vi "Init Events.vi"(8 "error in (no error)":errorcluster, 11 "TSEngine in":refnum<class "Engine.lvclass">) -> (0 "error out":errorcluster, 3 "TSEngine out":refnum<class "Engine.lvclass">, 4 "Event Reg":refnum<event-registration>, 6 "Events":T1)   [LabVIEW 2020, in "TSS.lvlib" / "Engine.lvclass"]
uses:
  Engine.lvclass
  Events.ctl
  Create VC Event Data.ctl
  Variable Container Type.ctl
  VariableContainer/Typedefs/Session Handle.ctl
  VariableContainer/VariableContainer.lvclass
  Create Report Event Data.ctl
  Execution/Typedefs/Session Handle.ctl
  Execution/Execution.lvclass
  Report/Typedefs/Session Handle.ctl
  Report/Report.lvclass
  Open Sequence File Event Data.ctl
  Data Types/File Load Options.ctl
  SequenceFile/Typedefs/Session Handle.ctl
  SequenceFile/SequenceFile.lvclass
  Session Notification.ctl
  Prepare Execution Event Data.ctl
  Execution/Execution Options.ctl
  Engine.lvclass/Engine.ctl
  TSS.lvlib
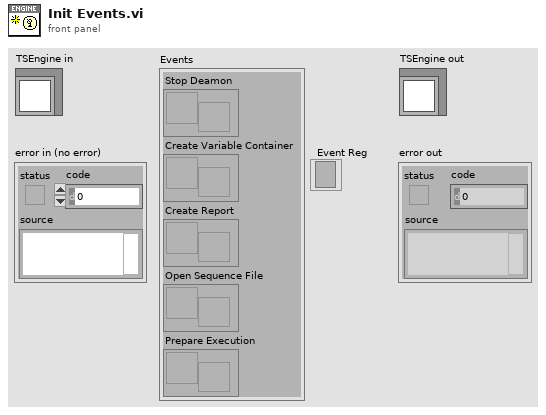
[diagram p1: front panel]
types:
  T1 = typedef "TSS.lvlib/Engine.lvclass/Events.ctl" = cluster{"Stop Deamon":refnum<user-event>, "Create Variable Container":refnum<user-event>, "Create Report":refnum<user-event>, "Open Sequence File":refnum<user-event>, "Prepare Execution":refnum<user-event>}
  T2 = typedef "TSS.lvlib/Engine.lvclass/Prepare Execution Event Data.ctl" = cluster{"Execution Options":T3, "Engine":refnum<data-value>, "Session Notifier":refnum<notifier>}
  T3 = typedef "TSS.lvlib/Execution.lvclass/Execution Options.ctl" = cluster{"Use Default Model":bool}
  T4 = typedef "TSS.lvlib/Engine.lvclass/Open Sequence File Event Data.ctl" = cluster{"File Path":path, "Load Options":T5, "Current Seq File (None)":T6, "Session Notifier":refnum<notifier>, "Engine":refnum<data-value>}
  T5 = typedef "TSS.lvlib/File Load Options.ctl" = cluster{"Use Search Dirs? (T)":bool, "Conflict as Error? (T)":bool, "Check Station Model? (F)":bool, "Preload Modules? (T)":bool, "Skip Load Callback? (F)":bool, "Reload if Loaded? (F)":bool}
  T6 = typedef "TSS.lvlib/SequenceFile.lvclass/Session Handle.ctl" = refnum<data-value>
  T7 = typedef "TSS.lvlib/Engine.lvclass/Create Report Event Data.ctl" = cluster{"Execution":T8, "Report Notifier":refnum<notifier>}
  T8 = typedef "TSS.lvlib/Execution.lvclass/Session Handle.ctl" = refnum<data-value>
  T9 = typedef "TSS.lvlib/Engine.lvclass/Create VC Event Data.ctl" = cluster{"Type":T10, "Notifier":refnum<notifier>}
  T10 = typedef "TSS.lvlib/Engine.lvclass/Variable Container Type.ctl" = enum16{"StationGlobals", "TemporaryGlobals", "NewPropertyObject"}
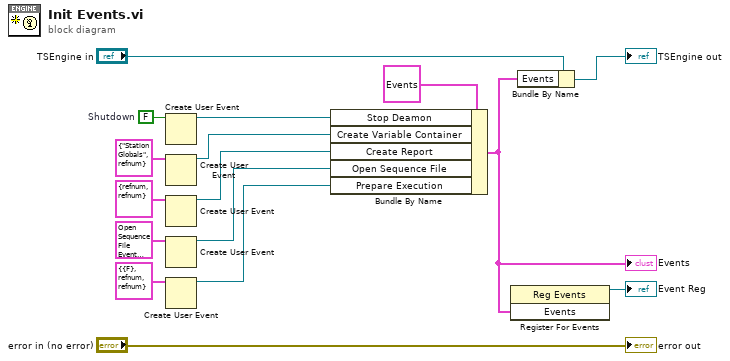
[diagram p0: block diagram]
diagram:
  w15 = FALSE  # Shutdown
  n1 = Create User Event(user event datatype=w15) -> (user event=w11:refnum<user-event>)  [unwired: 1 in, 1 out]
  n2 = Create User Event(user event datatype=T9 {"Type"=enum."StationGlobals", "Notifier"=refnum} ("Create VariableContainer Session")) -> (user event=w10:refnum<user-event>)  [unwired: 1 in, 1 out]
  n3 = Create User Event(user event datatype=T7 {"Execution"=refnum, "Report Notifier"=refnum} ("Create Report Event Data")) -> (user event=w5:refnum<user-event>)  [unwired: 1 in, 1 out]
  n4 = Create User Event(user event datatype=T4 {"File Path"=path "", "Load Options"={"Use Search Dirs? (T)"=FALSE, "Conflict as Error? (T)"=FALSE, "Check Station Model? (F)"=FALSE, "Preload Modules? (T)"=FALSE, "Skip Load Callback? (F)"=FALSE, "Reload if Loaded? (F)"=FALSE}, "Current Seq File (None)"=refnum, "Session Notifier"=refnum, "Engine"=refnum} ("Open Sequence File Event Data")) -> (user event=w3:refnum<user-event>)  [unwired: 1 in, 1 out]
  n5 = Create User Event(user event datatype=T2 {"Execution Options"={"Use Default Model"=FALSE}, "Engine"=refnum, "Session Notifier"=refnum} ("Prepare Execution Event Data")) -> (user event=w1:refnum<user-event>)  [unwired: 1 in, 1 out]
  n6 = Bundle By Name(cluster=T1 {"Stop Deamon"=refnum, "Create Variable Container"=refnum, "Create Report"=refnum, "Open Sequence File"=refnum, "Prepare Execution"=refnum} ("Events"), "Stop Deamon"=w11, "Create Variable Container"=w10, "Create Report"=w5, "Open Sequence File"=w3, "Prepare Execution"=w1) -> (w8:T1)
  "Events" <- w8
  n7 = register-events(w8) -> (reference out=→"Event Reg":refnum<event-registration>)  [unwired: 2 in, 1 out]
  n8 = Bundle By Name(cluster="TSEngine in", "Events"=w8) -> (→"TSEngine out":refnum<class "Engine.lvclass">)
  "error out" <- "error in (no error)"
